vi "Password Authentication.vi"(5 "Username":string, 6 "Password":string, 7 "Address":string, 8 "Error In":errorcluster) -> (0 "Error Out":errorcluster)   [LabVIEW 2018, in "Tests.lvlib" / "Session.lvlib"]
uses:
  Session.lvlib
  src/Toolkit/Session/Support/Create from SSH.vi
  src/Toolkit/Session/Support/Destroy to SSH.vi
  <vilib>/addons/_JKI Toolkits/Caraya/classes/Test/Test.lvclass
  src/Toolkit/SSH/SSH.lvclass
  src/Toolkit/Session/Session.lvclass
  <vilib>/addons/_JKI Toolkits/Caraya/classes/Assert/Assert.lvclass
  Tests.lvlib
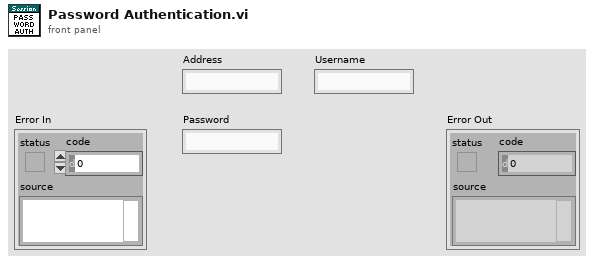
[diagram p1: front panel]
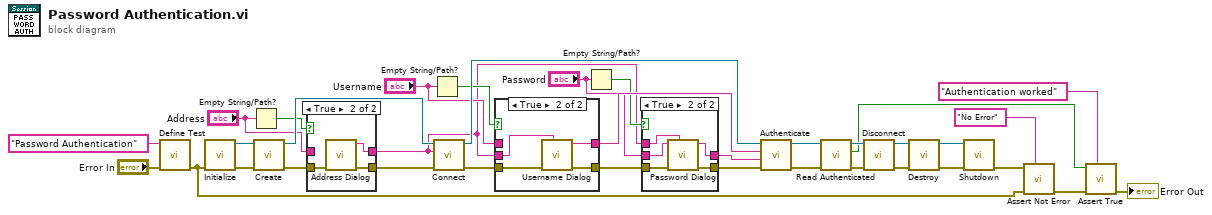
[diagram p0: block diagram]
diagram:
  n1 = call <vilib>:"Define Test.vi"("error in (no error)"="Error In", "Label (VI Title)"="Password Authentication") -> ("error out"=w27:errorcluster)  [unwired: 9 in]
  n2 = call "Initialize.vi"("Error In"=w27) -> ("Error Out"=w33:errorcluster, "SSH"=w32:refnum<class "SSH.lvclass">)  [unwired: 9 in]
  n3 = Empty String/Path?(string/path="Address") -> (empty?=w14:bool)
  n4 = call-poly "Create.vi"("Error In"=w33, "SSH"=w32) -> ("Error Out"=w12:errorcluster, "Sesssion"=w25:refnum<class "Session.lvclass">)  [unwired: 8 in]
  n5 = case shown="True" w14 {
    tunnel: w12 -> [w36 w40]
    tunnel: [w36 w39] -> w11
    tunnel: [w37 w38] -> w1
    tunnel: "Address" -> [w37 _]
    frame False {
    }
    frame True {
      n6 = call "Address Dialog.vi"("Error In"=w40) -> ("Error Out"=w39:errorcluster, "Address Out"=w38:string)  [unwired: 9 in]
    }
  }
  n7 = Empty String/Path?(string/path="Username") -> (empty?=w9:bool)
  n8 = call "Connect.vi"("Error In"=w11, "Address"=w1, "Session In"=w25) -> ("Error Out"=w10:errorcluster, "Sesssion Out"=w22:refnum<class "Session.lvclass">)  [unwired: 7 in]
  n9 = case shown="True" w9 {
    tunnel: w10 -> [w42 w46]
    tunnel: [w41 w45] -> w8
    tunnel: [w42 w44] -> w4
    tunnel: "Username" -> [w41 _]
    tunnel: w1 -> [_ w43]
    frame False {
    }
    frame True {
      n10 = call "Username Dialog.vi"("Address"=w43, "Error In"=w46) -> ("Error Out"=w44:errorcluster, "Username Out"=w45:string)  [unwired: 8 in]
    }
  }
  n11 = Empty String/Path?(string/path="Password") -> (empty?=w5:bool)
  n12 = case shown="True" w5 {
    tunnel: "Password" -> [w48 w53]
    tunnel: w4 -> [w47 w52]
    tunnel: [w47 w51] -> w3
    tunnel: [w48 w50] -> w2
    tunnel: w1 -> [_ w49]
    frame False {
    }
    frame True {
      n13 = call "Password Dialog.vi"("Address"=w49, "Error In"=w52, "Password In"=w53) -> ("Error Out"=w51:errorcluster, "Password Out"=w50:string)  [unwired: 7 in]
    }
  }
  n14 = call-poly "Authenticate.vi"("Error In"=w3, "Password"=w2, "Username"=w8, "Session In"=w22) -> ("Error Out"=w20:errorcluster, "Sesssion Out"=w21:refnum<class "Session.lvclass">)  [unwired: 6 in]
  n15 = call "Read Authenticated.vi"("Error In"=w20, "Session In"=w21) -> ("Error Out"=w19:errorcluster, "Authenticated"=w16:bool, "Sesssion Out"=w18:refnum<class "Session.lvclass">)  [unwired: 7 in]
  n16 = call "Disconnect.vi"("Error In"=w19, "Session In"=w18) -> ("Error Out"=w23:errorcluster, "Sesssion Out"=w24:refnum<class "Session.lvclass">)  [unwired: 8 in]
  n17 = call-poly "Destroy.vi"("Error In"=w23, "Session"=w24) -> ("Error Out"=w30:errorcluster, "SSH"=w31:refnum<class "SSH.lvclass">)  [unwired: 8 in]
  n18 = call "Shutdown.vi"("Error In"=w30, "SSH"=w31) -> ("Error Out"=w29:errorcluster)  [unwired: 9 in]
  n19 = call <vilib>:"Assert Not Error.vi"("Label"="No Error", "error in (no error)"=w27, "Not Error?"=w29) -> ("error out"=w26:errorcluster)  [unwired: 8 in]
  n20 = call <vilib>:"Assert True.vi"("Label"="Authentication worked", "error in (no error)"=w26, "True?"=w16) -> ("error out"=→"Error Out":errorcluster)  [unwired: 8 in]
